vi "Parse Error XML.vi"(9 "Code Tag Value":string, 10 "Error XML":string, 11 "AWS Core":refnum<class "HTTP Request.lvclass">) -> (1 "Error Description Override":string, 2 "Error Code":i32, 3 "Warning":bool)   [LabVIEW 2015, in "NI_AWS_Core.lvlib" / "HTTP Request.lvclass"]
uses:
  HTTP Request.lvclass
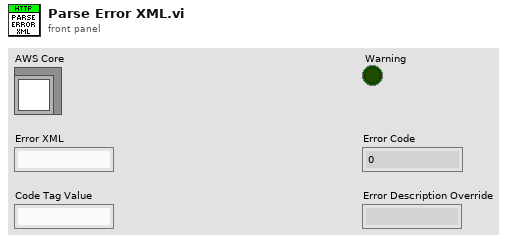
[diagram p1: front panel]
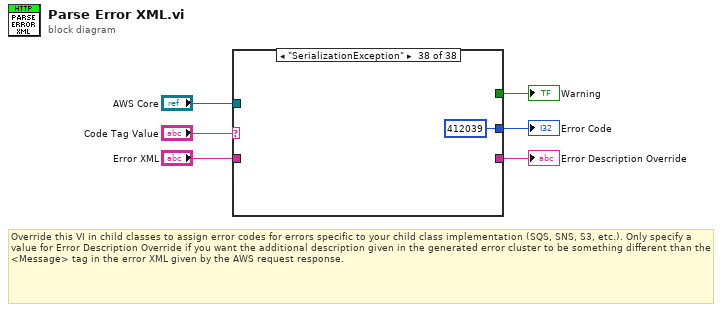
[diagram p0: block diagram]
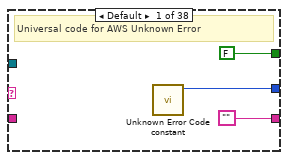
[diagram p2: hidden frame]
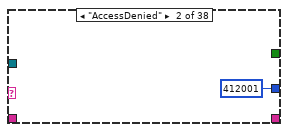
[diagram p3: hidden frame]
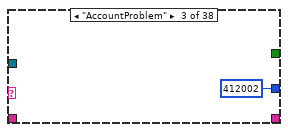
[diagram p4: hidden frame]
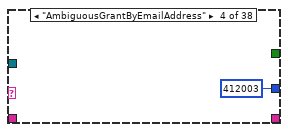
[diagram p5: hidden frame]
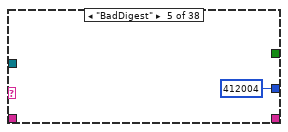
[diagram p6: hidden frame]
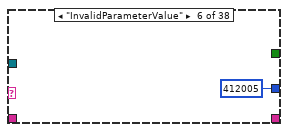
[diagram p7: hidden frame]
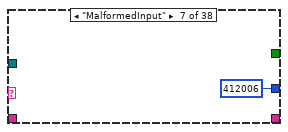
[diagram p8: hidden frame]
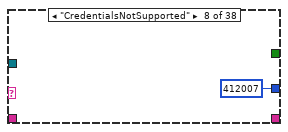
[diagram p9: hidden frame]
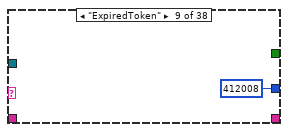
[diagram p10: hidden frame]
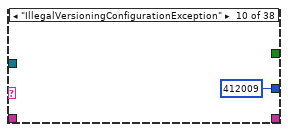
[diagram p11: hidden frame]
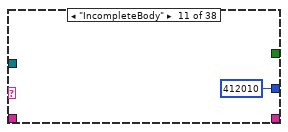
[diagram p12: hidden frame]
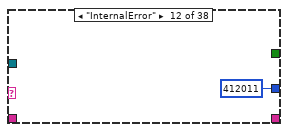
[diagram p13: hidden frame]
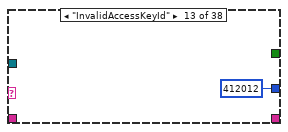
[diagram p14: hidden frame]
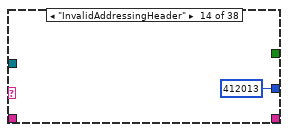
[diagram p15: hidden frame]
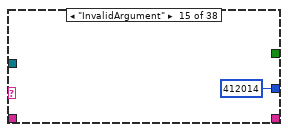
[diagram p16: hidden frame]
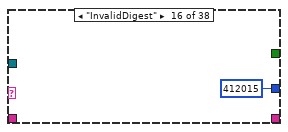
[diagram p17: hidden frame]
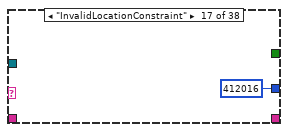
[diagram p18: hidden frame]
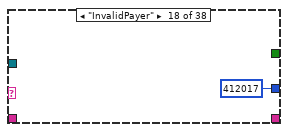
[diagram p19: hidden frame]
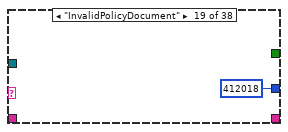
[diagram p20: hidden frame]
diagram:
  # "Override this VI in child classes to assign error codes for errors specific to your child class implementation (SQS, SNS, S3, etc.). Only specify a value for Error Description Override if you want the additional description given in the generated error cluster to be something different than the <Message> tag in the error XML given by the AWS request response."
  n1 = case shown="\"SerializationException\"" "Code Tag Value" {
    tunnel: [w7 412001 412002 412003 412004 412005 412006 412007 412008 412009 412010 412011 412012 412013 412014 412015 412016 412017 412018 412019 412020 412021 412022 412023 412024 412025 412026 412027 412028 412029 412030 412031 412032 412033 412034 412037 412038 412039] -> w2
    tunnel: [FALSE _ _ _ _ _ _ _ _ _ _ _ _ _ _ _ _ _ _ _ _ _ _ _ _ _ _ _ TRUE _ _ _ _ TRUE TRUE _ _ _] -> w3
    tunnel: "Error XML" -> [_ _ _ _ _ _ _ _ _ _ _ _ _ _ _ _ _ _ _ _ _ _ _ _ _ _ _ _ _ _ _ _ _ _ _ _ _ _]
    tunnel: ["" _ _ _ _ _ _ _ _ _ _ _ _ _ _ _ _ _ _ _ _ _ _ _ _ _ _ _ _ _ _ _ _ _ _ _ _ _] -> w4
    tunnel: "AWS Core" -> [_ _ _ _ _ _ _ _ _ _ _ _ _ _ _ _ _ _ _ _ _ _ _ _ _ _ _ _ _ _ _ _ _ _ _ _ _ _]
    frame Default {
      # "Universal code for AWS Unknown Error"
      n2 = call "Unknown Error Code constant.vi"() -> ("AWS Unknown Error Code value"=w7:i32)  [unwired: 11 in]
    }
    frame "AccessDenied" {
    }
    frame "AccountProblem" {
    }
    frame "AmbiguousGrantByEmailAddress" {
    }
    frame "BadDigest" {
    }
    frame "InvalidParameterValue" {
    }
    frame "MalformedInput" {
    }
    frame "CredentialsNotSupported" {
    }
    frame "ExpiredToken" {
    }
    frame "IllegalVersioningConfigurationException" {
    }
    frame "IncompleteBody" {
    }
    frame "InternalError" {
    }
    frame "InvalidAccessKeyId" {
    }
    frame "InvalidAddressingHeader" {
    }
    frame "InvalidArgument" {
    }
    frame "InvalidDigest" {
    }
    frame "InvalidLocationConstraint" {
    }
    frame "InvalidPayer" {
    }
    frame "InvalidPolicyDocument" {
    }
    frame "InvalidSecurity" {
    }
    frame "InvalidToken" {
    }
    frame "InvalidURI" {
    }
    frame "MalformedXML" {
    }
    frame "MethodNotAllowed" {
    }
    frame "NoSuchVersion" {
    }
    frame "NotImplemented" {
    }
    frame "OperationAborted" {
    }
    frame "PreconditionFailed" {
    }
    frame "Redirect" {
    }
    frame "RequestTimeout" {
    }
    frame "RequestTimeTooSkewed" {
    }
    frame "SignatureDoesNotMatch" {
    }
    frame "SlowDown" {
    }
    frame "TemporaryRedirect" {
    }
    frame "Throttled", "Throttling" {
    }
    frame "ValidationError" {
    }
    frame "InvalidParameter" {
    }
    frame "SerializationException" {
    }
  }
  "Error Description Override" <- w4
  "Warning" <- w3
  "Error Code" <- w2
